vi "VHistory - Get Arbitrary Variable History.vi"(4 "reverse order (T)":bool=TRUE, 6 "mode":u32(ring) items=["TimeRange", "N-Vals", "NewVals"], 7 "VC Handle":T1=-1, 8 "error in":errorcluster, 9 "time range (all)":cluster{"t1":dbl, "t2":dbl} {"t2" format="%<%H:%M:%S%2u\n%d/%m/%Y>T"; "t1" format="%<%H:%M:%S%2u\n%d/%m/%Y>T"}, 10 "N vals (all)":i32=-1, 11 "name_spec":string) -> (0 "error out":errorcluster, 1 "history":string[](array[string]), 2 "time stamps":dbl[](array[numeric]) format="%<%H:%M:%S%2u\n%d/%m/%Y>T", 3 "dup name_spec":string, 5 "writer IDs":u32[](array[numeric]))   [LabVIEW 2021]
doc: "This VI returns the history of a variable of an arbitrary data type; both predefined and user-defined data types are supported. Refer to the VI help for more details.\n\n<b>VC Handle</b> and <b>name_spec</b> controls specify the desired variable. The variable must exist and have a history attached; otherwise, the VI returns an error. Use <b>VHistory - History Controller.vi</b> to attach a history to a variable.\n\n<b>VC Handle</b> specifies the handle of the variable context. To operate on a global variable, pass -1 to this input. This input is ignored if the <b>name_spec</b> control refers to a variable by an alias.\n\n<b>name_spec</b> is the name specifier of the desired variable. Usually, it is merely a variable name; however, its generic format is '[name][=alias]', where either 'name' or '=alias' can be omitted but not both.\n\n<b>mode</b> control specifies the method used to retrieve the history:\n 'TimeRange' : returns history values that fall within the specified <b>time range</b>.\n 'N-Vals' : returns the most recent <b>N Vals</b> values stored in the history.\n 'NewVals' : returns values added to the history since the last call to this VI in 'NewVals' mode.\n\n<b>reverse order</b> control specifies whether the history is returned in reverse (TRUE) or direct (FALSE) chronological order.\n\n<b>N Vals</b> control is only used in 'N-Vals' mode. If <b>N Vals</b> is less than zero (default), the VI returns the complete stored history of the specified variable. Otherwise, the VI returns only the most recent <b>N Vals</b> values.\n\n<b>time range</b> control is only used in 'TimeRange' mode. If both the t1 and t2 members of <b>time range</b> are equal to zero (default), the VI returns the complete stored history of the specified variable. Otherwise, the VI returns only values that have timestamps in the range from Min(t1,t2) to Max(t1,t2).\n\n<b>history</b> indicator returns the history values represented in the Flattened-To-String format.\n\n<b>time stamps</b> indicator returns the timestamps, in the standard LabVIEW date/time format, of the respective elements in <b>history</b>.\n\n<b>writer IDs</b> indicator returns the IDs of the writers for the respective elements in <b>history</b>. If the history does not store writer IDs, this indicator returns an empty array.\n\n::: CalcExpress Toolkit :::\nCopyright (c) 2000-2026 Konstantin Shifershteyn. All rights reserved."
uses:
  cetypes.llb/VarMan Variable Context Handle.ctl
  cersrc/celveng32.dll
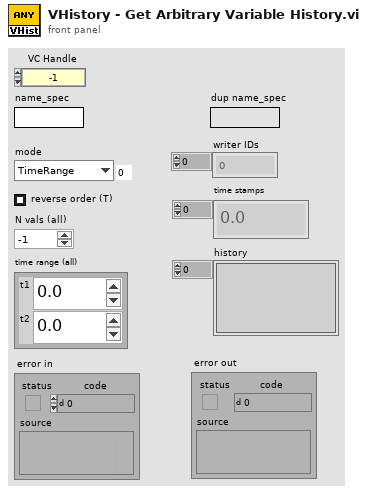
[diagram p1: front panel]
types:
  T1 = typedef "VarMan Variable Context Handle.ctl" = i32
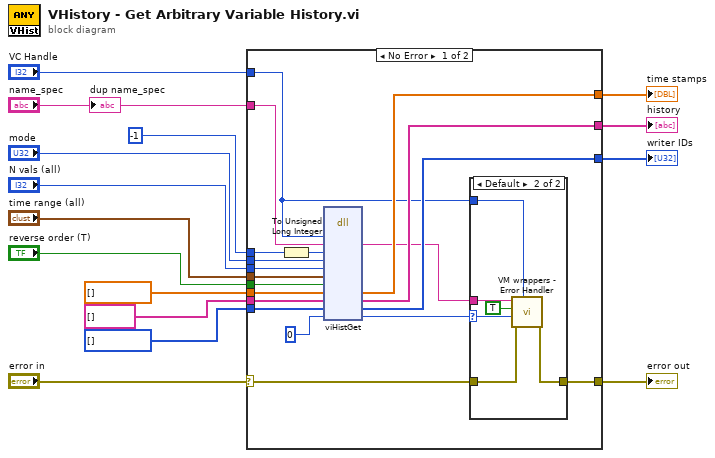
[diagram p0: block diagram]
diagram:
  n1 = case shown="No Error" "error in" {
    selector: "error in" -> [w19 w42]
    tunnel: -1 -> [w34 _]
    tunnel: [w33 w42] -> w5
    tunnel: "VC Handle" -> [w16 _]
    tunnel: "name_spec" -> [w32 _]
    tunnel: "mode" -> [w30 _]
    tunnel: "N vals (all)" -> [w29 _]
    tunnel: "time range (all)" -> [w28 _]
    tunnel: "reverse order (T)" -> [w27 _]
    tunnel: dbl[] [] ("time stamps") -> [w26 _]
    tunnel: string[] [] ("history") -> [w25 _]
    tunnel: [w23 _] -> w2
    tunnel: [w22 _] -> w3
    tunnel: u32[] [] ("history") -> [w21 _]
    tunnel: [w20 _] -> w4
    frame No Error {
      n2 = To Unsigned Long Integer(number=w34) -> (unsigned 32bit integer=w31:u32)
      n3 = dll-call lib="C:/LV Projects/CalcExpress 40 LV2021/vi.lib/addons/CalcExpress/cersrc/celveng*.dll" fn="viHistGet"("vch"=w16, "name"=w32, "type"=w31, "mode"=w30, "nvals"=w29, "tRange"=w28, "rev"=w27, "time"=w26, "data"=w25, "writerIDs"=w21, "errc"=u16 0) -> ("name"=w17:string, "time"=w23:dbl[], "data"=w22:string[], "writerIDs"=w20:u32[], "errc"=w18:u16)  [unwired: 10 in, 2 out]
      n4 = case shown="Default" w18 {
        selector: w18 -> [_ w37]
        tunnel: w19 -> [w35 w41]
        tunnel: w17 -> [_ w40]
        tunnel: [w35 w39] -> w33
        tunnel: w16 -> [_ w36]
        frame 0 {
        }
        frame Default {
          n5 = call "VM wrappers - Error Handler.vi"("VC Handle"=w36, "error before"=w41, "VarMan error"=w37, "show name spec (F)"=TRUE, "name spec"=w40) -> ("error out"=w39:errorcluster)  [unwired: 5 in, 1 out]
        }
      }
    }
    frame Error {
    }
  }
  "time stamps" <- w2
  "error out" <- w5
  "history" <- w3
  "writer IDs" <- w4
  "dup name_spec" <- "name_spec"
